vi "PrintHello.vi"(8 "error in (no error)":errorcluster, 11 "ProductA in":refnum<class "ProductA.lvclass">) -> (0 "error out":errorcluster, 3 "ProductA out":refnum<class "ProductA.lvclass">)   [LabVIEW 2018, in "ProductA.lvclass"]
uses:
  ProductA.lvclass
  ConsoleOut/Print Options.ctl
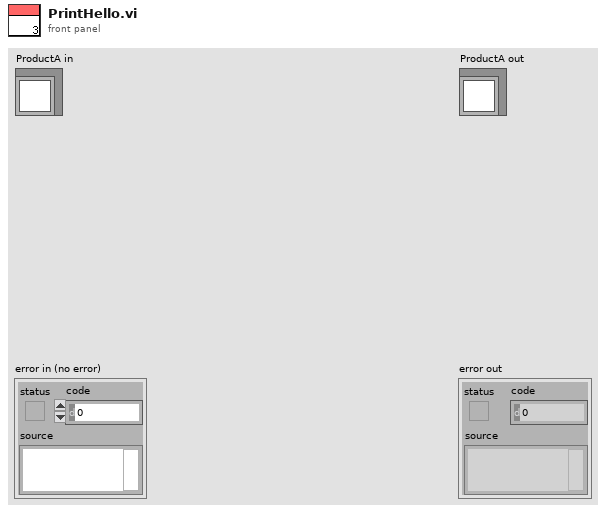
[diagram p1: front panel]
types:
  T1 = typedef "Print Options.ctl" = enum16{"Create", "Get Reference", "Print", "Print Header", "Close"}
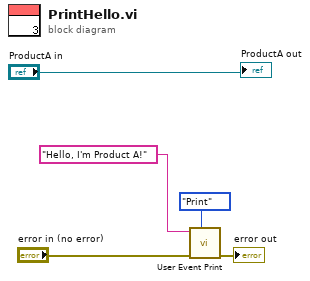
[diagram p0: block diagram]
diagram:
  n1 = call "User Event Print.vi"("Options"=Print_Options."Print", "error in (no error)"="error in (no error)", "String to Print"="Hello, I'm Product A!" ("message")) -> ("error out"=→"error out":errorcluster)  [unwired: 7 in, 1 out]
  "ProductA out" <- "ProductA in"
